vi "Name Value Organize Tags.vi"(0 "Name Values":string[][][](array[string]), 7 "Group Names":string[](array[string]), 11 "Notes":string) -> (4 "Name Value Group":string[][](array[string]))   [LabVIEW 2020]
panel:
  in  "Notes 2":string
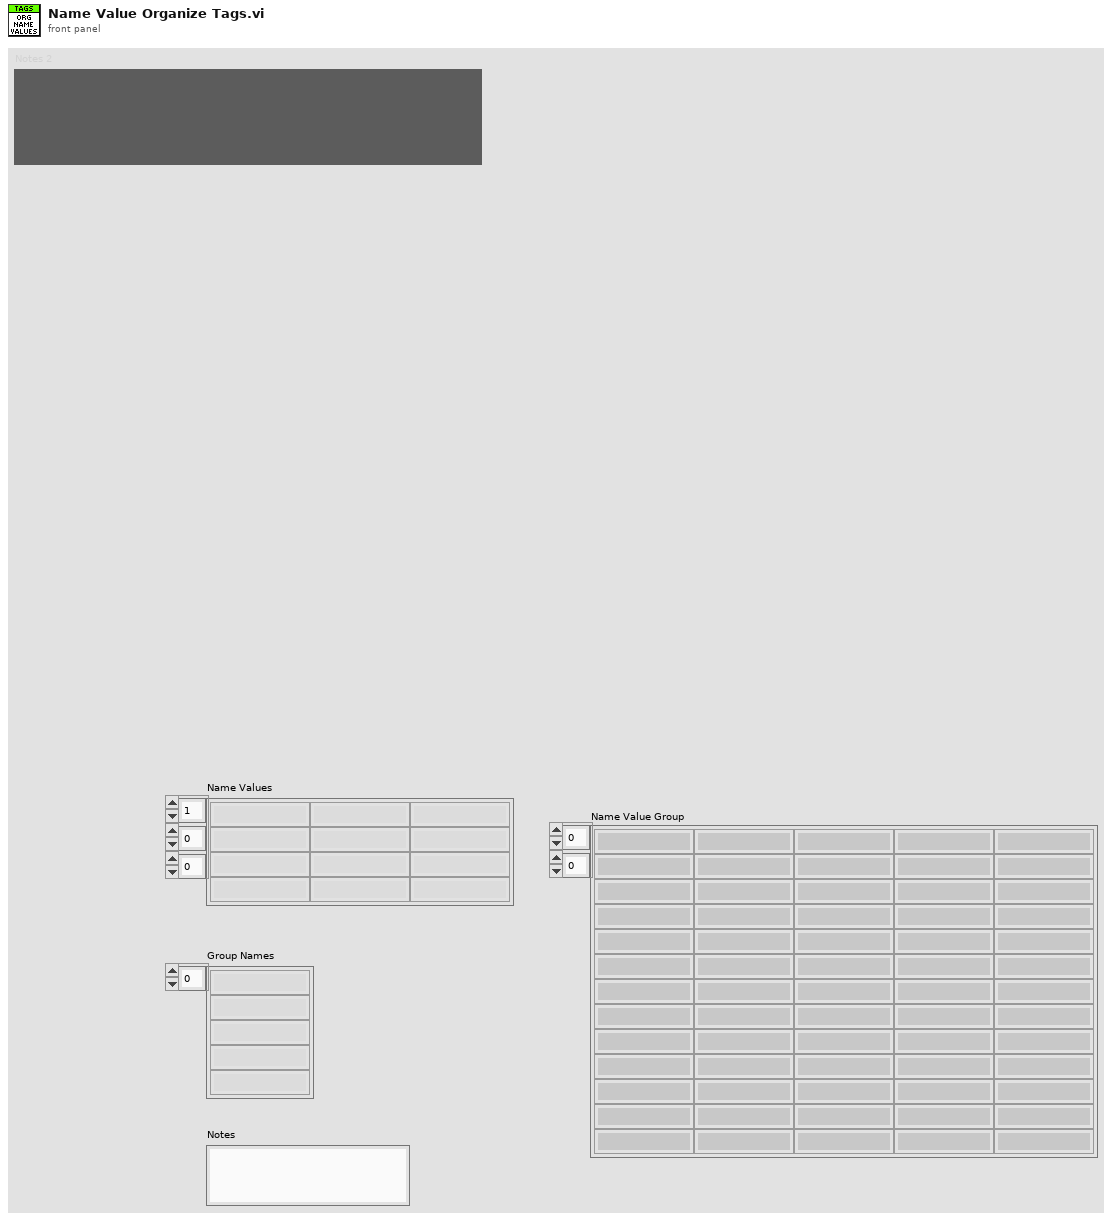
[diagram p1: front panel]
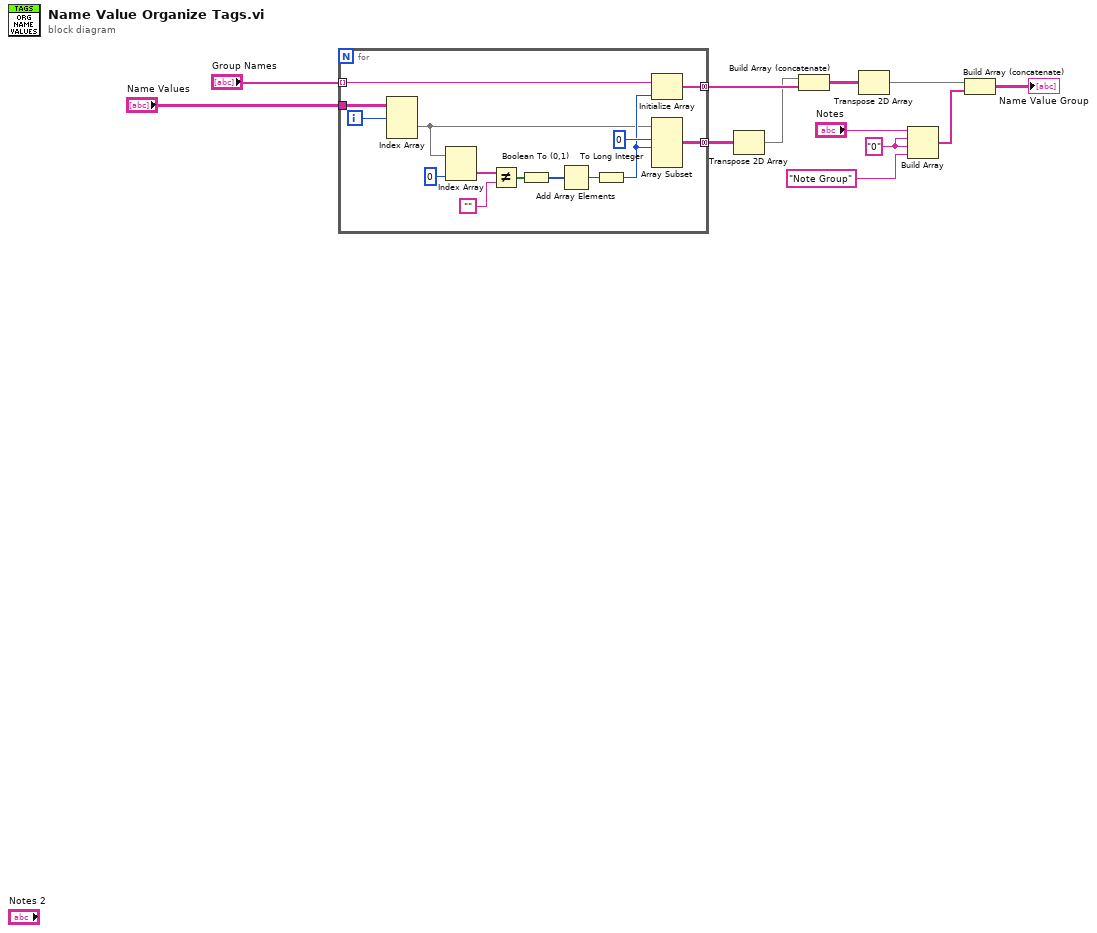
[diagram p0: block diagram]
diagram:
  w12 = "0" ("element")
  n1 = for {
    tunnel: "Group Names" -> [w21] mode=indexing
    tunnel: [w14] -> w9 mode=concatenating
    tunnel: [w15] -> w8 mode=concatenating
    tunnel: "Name Values" -> [w13]
    i -> [w19]
    n2 = Index Array(array=w13, index (dim 0)=w19) -> (element=w18:string[][])  [unwired: 2 in]
    n3 = Index Array(array=w18, index (col)=0 ("disabled index (col)")) -> (element=w16:string[])  [unwired: 1 in]
    n4 = Not Equal?(x=w16, y="") -> (x != y?=w25:bool[])
    n5 = Boolean To (0,1)(Boolean=w25) -> (0, 1=w24:i16[])
    n6 = Add Array Elements(numeric array=w24) -> (sum=w23:i16)
    n7 = To Long Integer(number=w23) -> (32bit integer=w20:i32)
    n8 = Initialize Array(w21, w20) -> (w15:string[])
    n9 = Array Subset(array=w18, index (row)=0 ("index"), length (row)=w20) -> (w14:string[][])  [unwired: 2 in]
  }
  n10 = Transpose 2D Array(2D array=w9) -> (transposed array=w3:string[][])
  n11 = Build Array (concatenate)(w3, w8) -> (w2:string[][])
  n12 = Transpose 2D Array(2D array=w2) -> (transposed array=w1:string[][])
  n13 = Build Array("Notes", w12, w12, "Note Group" ("string")) -> (w10:string[])
  n14 = Build Array (concatenate)(w1, w10) -> (→"Name Value Group":string[][])
